vi "Create DAQmx Tasks.vi"(8 "Error In":errorcluster, 11 "Daqmx Module configuration":refnum<class "Daqmx Module configuration.lvclass">) -> (0 "Error Out":errorcluster, 2 "DAQ Tasks":T1)   [LabVIEW 2015, in "DAQmx Module Runtime.lvclass"]
doc: "Create unique tasks to be used in DCAF DAQmx module. Task names are based on module's UID and task type."
uses:
  DAQmx Module Runtime.lvclass
  DAQ Tasks.ctl
  configuration/Daqmx Module configuration.lvclass
  <vilib>/NI/Configuration Framework/serializable configuration/NISE_CEF_serializable configuration.lvclass/NISE_CEF_serializable configuration.ctl
  <vilib>/Utility/LVClass/Get LV Class Name.vi
  <vilib>/NI/Configuration Framework/error generator/NISE_error generator.vi
  <vilib>/NI/Configuration Framework/serializable configuration/NISE_CEF_serializable configuration.lvclass
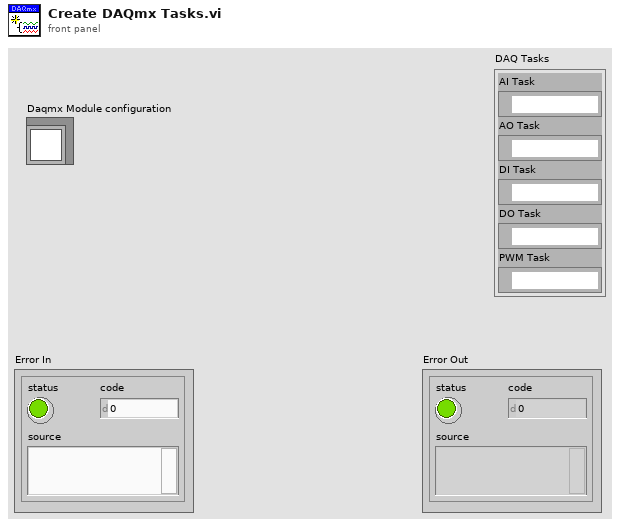
[diagram p1: front panel]
types:
  T1 = typedef "DAQmx Module Runtime.lvclass/DAQ Tasks.ctl" = cluster{"AI Task":refnum<k21>, "AO Task":refnum<k21>, "DI Task":refnum<k21>, "DO Task":refnum<k21>, "PWM Task":refnum<k21>}
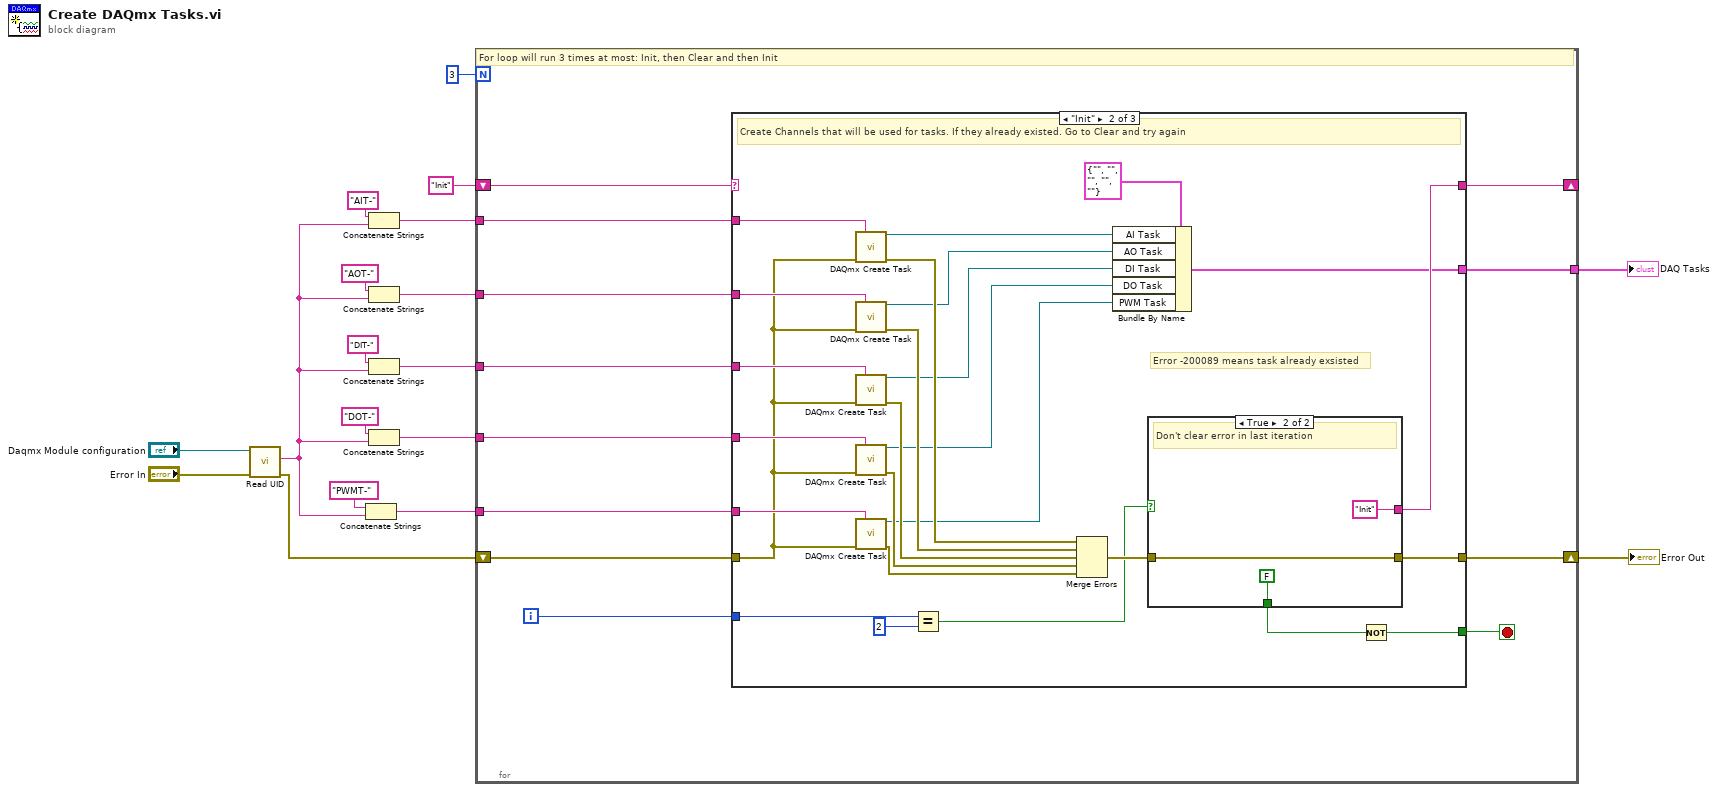
[diagram p0: block diagram]
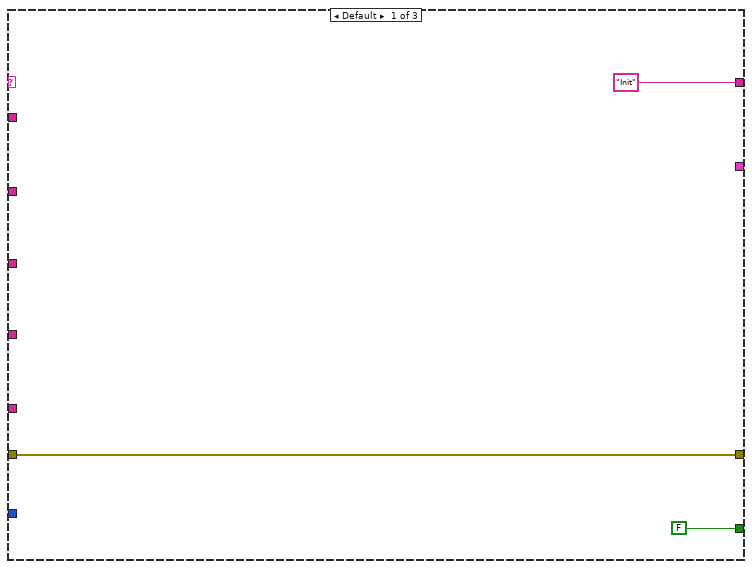
[diagram p2: hidden frame]
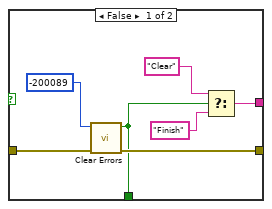
[diagram p3: hidden frame]
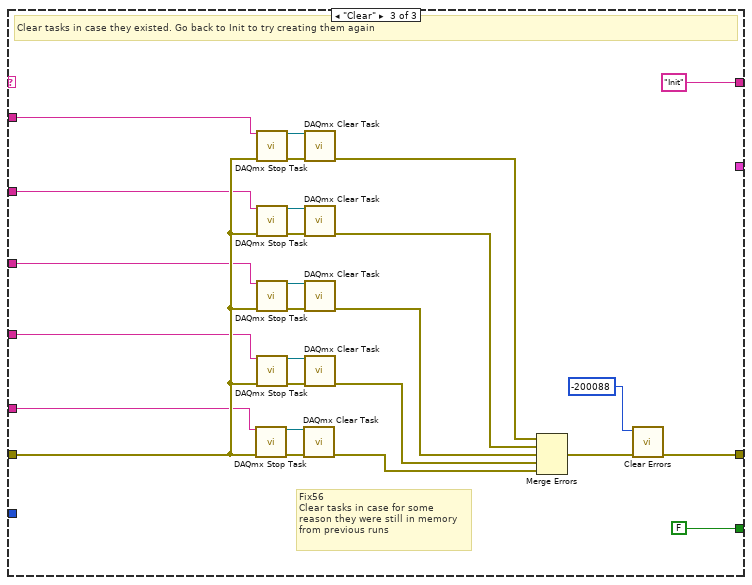
[diagram p4: hidden frame]
diagram:
  n1 = call <vilib>:"Read UID.vi"("error in"="Error In", "configuration in"="Daqmx Module configuration") -> ("error out"=w8:errorcluster, "instance id"=w11:string)  [unwired: 7 in, 1 out]
  n2 = Concatenate Strings("PWMT-" ("new task name"), w11) -> (w7:string)
  n3 = Concatenate Strings("AIT-" ("new task name"), w11) -> (w3:string)
  n4 = Concatenate Strings("AOT-" ("new task name"), w11) -> (w4:string)
  n5 = Concatenate Strings("DIT-" ("new task name"), w11) -> (w5:string)
  n6 = Concatenate Strings("DOT-" ("new task name"), w11) -> (w6:string)
  n7 = for {
    N: 3 -> [_]
    tunnel: w3 -> [w29]
    tunnel: w4 -> [w28]
    tunnel: w5 -> [w27]
    tunnel: w6 -> [w26]
    tunnel: w7 -> [w25]
    shift-right: [w30] -> w2
    shift-left: w8 -> [w22]
    shift-right: [w23] -> _
    shift-left: "Init" -> [w24]
    tunnel: [w19] -> w1
    i -> [w20]
    stop <- w21 stop-if-true
    # "For loop will run 3 times at most: Init, then Clear and then Init"
    n8 = case shown="\"Init\"" w24 {
      tunnel: [w32 w48 w75] -> w30
      tunnel: w29 -> [_ w54 w74]
      tunnel: w28 -> [_ w53 w73]
      tunnel: w27 -> [_ w52 w72]
      tunnel: w26 -> [_ w51 w71]
      tunnel: w25 -> [_ w50 w70]
      tunnel: ["Init" w47 "Init"] -> w23
      tunnel: w22 -> [w32 w46 w85]
      tunnel: [FALSE w44 FALSE] -> w21
      tunnel: w20 -> [_ w43 _]
      tunnel: [_ w34 _] -> w19
      frame Default {
      }
      frame "Init" {
        # "Error -200089 means task already exsisted"
        # "Create Channels that will be used for tasks. If they already existed. Go to Clear and try again"
        n9 = call <vilib>:"DAQmx Create Task.vi"("new task name"=w54, "error in"=w46) -> ("task out"=w39:refnum<k21>, "error out"=w57:errorcluster)  [unwired: 12 in]
        n10 = call <vilib>:"DAQmx Create Task.vi"("new task name"=w53, "error in"=w46) -> ("task out"=w38:refnum<k21>, "error out"=w58:errorcluster)  [unwired: 12 in]
        n11 = call <vilib>:"DAQmx Create Task.vi"("new task name"=w52, "error in"=w46) -> ("task out"=w37:refnum<k21>, "error out"=w59:errorcluster)  [unwired: 12 in]
        n12 = call <vilib>:"DAQmx Create Task.vi"("new task name"=w51, "error in"=w46) -> ("task out"=w36:refnum<k21>, "error out"=w55:errorcluster)  [unwired: 12 in]
        n13 = call <vilib>:"DAQmx Create Task.vi"("new task name"=w50, "error in"=w46) -> ("task out"=w35:refnum<k21>, "error out"=w56:errorcluster)  [unwired: 12 in]
        n14 = Equal?(x=w43, y=2) -> (x = y?=w41:bool)
        n15 = Merge Errors(w57, w58, w59, w55, w56) -> (w49:errorcluster)
        n16 = Bundle By Name(cluster=T1 {"AI Task"="", "AO Task"="", "DI Task"="", "DO Task"="", "PWM Task"=""} ("DAQ Tasks"), "AI Task"=w39, "AO Task"=w38, "DI Task"=w37, "DO Task"=w36, "PWM Task"=w35) -> (w34:T1)
        n17 = case shown="True" w41 {
          tunnel: w49 -> [w66 w67]
          tunnel: [w64 w67] -> w48
          tunnel: [w61 "Init"] -> w47
          tunnel: [w60 FALSE ("specific error cleared?")] -> w45
          frame False {
            n18 = call <vilib>:"Clear Errors.vi"("error in (no error)"=w66, "specific error code to clear (0: all)"=-200089) -> ("error out"=w64:errorcluster, "specific error cleared?"=w60:bool)  [unwired: 4 in]
            n19 = Select(t="Clear", s=w60, f="Finish") -> (s? t:f=w61:string)
          }
          frame True {
            # "Don't clear error in last iteration"
          }
        }
        n20 = Not(x=w45) -> (.not. x?=w44:bool)
      }
      frame "Clear" {
        # "Fix56\nClear tasks in case for some \nreason they were still in memory\nfrom previous runs"
        # "Clear tasks in case they existed. Go back to Init to try creating them again"
        n21 = call <vilib>:"DAQmx Stop Task.vi"("task/channels in"=w70, "error in"=w85) -> ("task out"=w87:refnum<k21>, "error out"=w86:errorcluster)  [unwired: 12 in]
        n22 = call <vilib>:"DAQmx Stop Task.vi"("task/channels in"=w74, "error in"=w85) -> ("task out"=w91:refnum<k21>, "error out"=w95:errorcluster)  [unwired: 12 in]
        n23 = call <vilib>:"DAQmx Stop Task.vi"("task/channels in"=w73, "error in"=w85) -> ("task out"=w90:refnum<k21>, "error out"=w92:errorcluster)  [unwired: 12 in]
        n24 = call <vilib>:"DAQmx Stop Task.vi"("task/channels in"=w72, "error in"=w85) -> ("task out"=w89:refnum<k21>, "error out"=w93:errorcluster)  [unwired: 12 in]
        n25 = call <vilib>:"DAQmx Stop Task.vi"("task/channels in"=w71, "error in"=w85) -> ("task out"=w88:refnum<k21>, "error out"=w94:errorcluster)  [unwired: 12 in]
        n26 = call <vilib>:"DAQmx Clear Task.vi"("task in"=w87, "error in"=w86) -> ("error out"=w78:errorcluster)  [unwired: 13 in]
        n27 = call <vilib>:"DAQmx Clear Task.vi"("task in"=w91, "error in"=w95) -> ("error out"=w83:errorcluster)  [unwired: 13 in]
        n28 = call <vilib>:"DAQmx Clear Task.vi"("task in"=w90, "error in"=w92) -> ("error out"=w82:errorcluster)  [unwired: 13 in]
        n29 = call <vilib>:"DAQmx Clear Task.vi"("task in"=w89, "error in"=w93) -> ("error out"=w81:errorcluster)  [unwired: 13 in]
        n30 = call <vilib>:"DAQmx Clear Task.vi"("task in"=w88, "error in"=w94) -> ("error out"=w80:errorcluster)  [unwired: 13 in]
        n31 = Merge Errors(w83, w82, w81, w80, w78) -> (w76:errorcluster)
        n32 = call <vilib>:"Clear Errors.vi"("error in (no error)"=w76, "specific error code to clear (0: all)"=-200088) -> ("error out"=w75:errorcluster)  [unwired: 4 in, 1 out]
      }
    }
  }
  "DAQ Tasks" <- w1
  "Error Out" <- w2
